vi "Get Size.vi"   [LabVIEW 2019, in "xy_utilities.lvlib"]
doc: "Get size of X and Y arrays.\n\nWire data to the data input to determine the polymorphic instance to use or manually select the instance."
uses:
  xy_utilities.lvlib
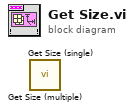
[diagram p0: block diagram]
diagram:
  n1 = call "Get Size (multiple).vi"() -> ()  [unwired: 8 in, 4 out]
  n2 = call "Get Size (single).vi"() -> ()  [unwired: 8 in, 4 out]
